vi "Data_Check.vi"(8 "error in (no error)":errorcluster, 9 "Refnum in":refnum<k21>) -> (0 "error out":errorcluster, 4 "disconnected?":bool)   [LabVIEW 2025]
uses:
  <resource>/objmgr/ni.dex.rc
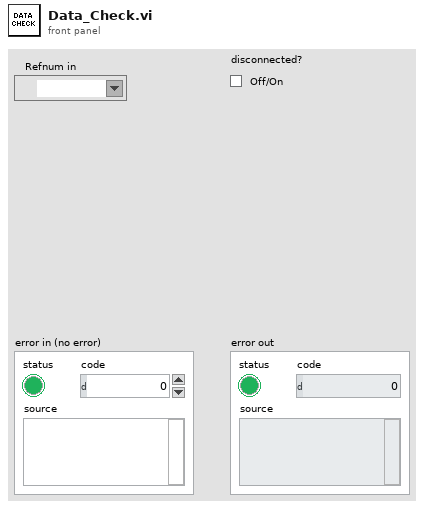
[diagram p1: front panel]
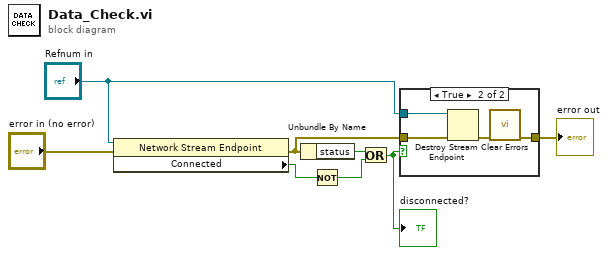
[diagram p0: block diagram]
diagram:
  n1 = property class="Network Stream Endpoint"(reference="Refnum in", error in="error in (no error)") -> (error out=w6:errorcluster, "Connected"=w3:bool)  [unwired: 1 out]
  n2 = Unbundle By Name(w6) -> ("status"=w5:bool)
  n3 = Not(x=w3) -> (.not. x?=w4:bool)
  n4 = Or(x=w5, y=w4) -> (x .or. y?=w1:bool)
  "disconnected?" <- w1
  n5 = case shown="True" w1 {
    tunnel: w6 -> [w9 w13]
    tunnel: [w9 w11] -> w7
    tunnel: "Refnum in" -> [_ w10]
    frame False {
    }
    frame True {
      n6 = Destroy Stream Endpoint(8:w13, 11:w10) -> (0:w12:errorcluster)
      n7 = call <vilib>:"Clear Errors.vi"("error in (no error)"=w12) -> ("error out"=w11:errorcluster)  [unwired: 5 in, 1 out]
    }
  }
  "error out" <- w7
